vi "CO monitor TurnTable.vi"(7 "error in (no error)":errorcluster caption="에러 입력(에러 없음)", 9 "Target Offset":dbl=2.0 format="%#_13g", 10 "Instrument Manager 입력":refnum<class "Instrument Manager.lvclass">) -> (0 "error out":errorcluster caption="에러 출력", 1 "In Offset Range?":bool, 2 "Current Angle":dbl, 3 "Instrument Manager 출력":refnum<class "Instrument Manager.lvclass">)   [LabVIEW 2023, in "Instrument Manager.lvclass"]
uses:
  Instrument Manager.lvclass
  Instrument Manager.lvclass/Instrument Manager.ctl
  Module/Turn Table and Mast Control/Interface Class/Turn Table/Interface - Turn Table.lvclass
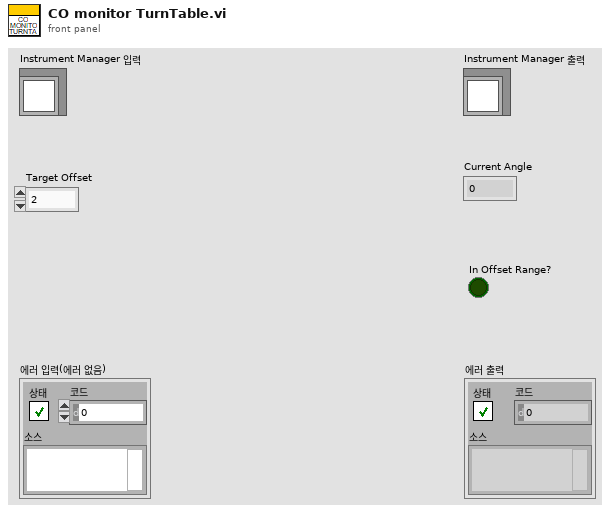
[diagram p1: front panel]
types:
  T1 = cluster{"Anritsu Call Box":refnum<class "Anritsu Call Box.lvclass">, "Spectrum Analyzer":refnum<class "Interface_Spectrum.lvclass">, "RF Switch Box":refnum<class "RF Filter Box.lvclass">, "Turn Table":refnum<class "Interface - Turn Table.lvclass">, "Mast":refnum<class "Interface - Mast.lvclass">, "3D Controller":refnum<class "Interface_3D Controller.lvclass">}
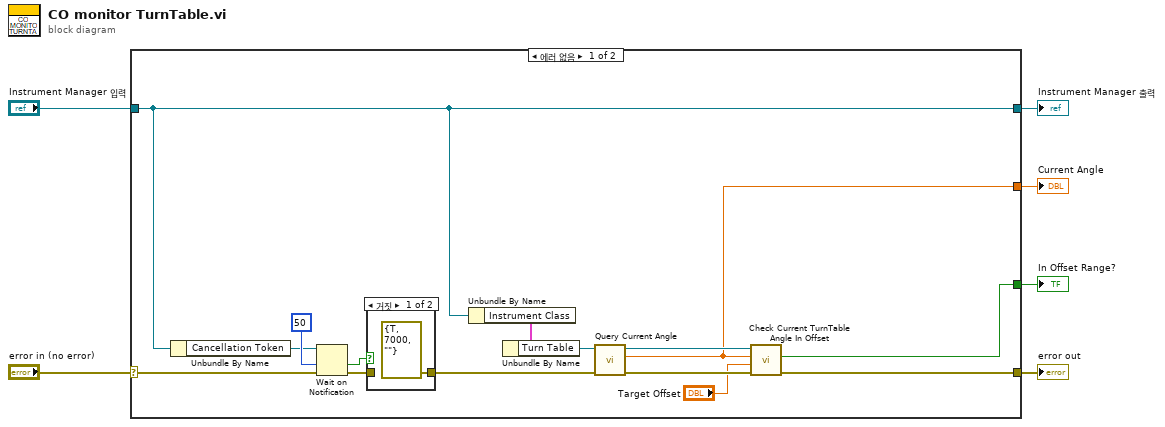
[diagram p0: block diagram]
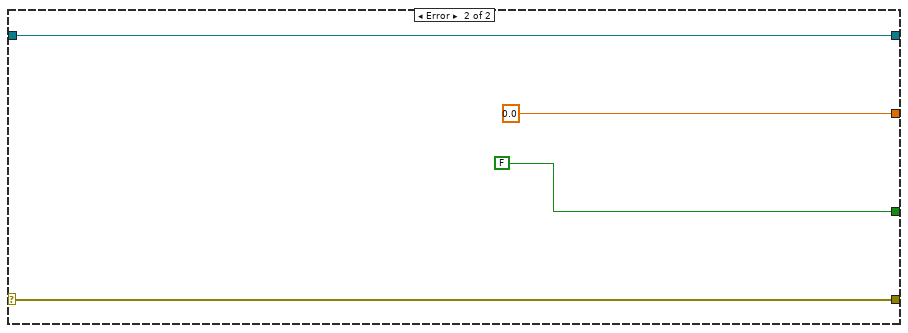
[diagram p3: hidden frame]
diagram:
  n1 = case shown="에러 없음" "error in (no error)" {
    selector: "error in (no error)" -> [w19 w27]
    tunnel: [w11 w27] -> w5
    tunnel: [w9 w26] -> w3
    tunnel: "Instrument Manager 입력" -> [w9 w26]
    tunnel: [w10 FALSE ("In Offset Range?")] -> w2
    tunnel: [w7 0.0 ("Current Angle")] -> w1
    frame No Error {
      n2 = Unbundle By Name(w9) -> ("Cancellation Token"=w8:refnum<notifier>)
      n3 = Wait on Notification(notifier=w8, timeout in ms (-1)=50 ("타임아웃(ms) (-1)"), error in (no error)=w19) -> (timed out?=w14:bool, error out=w13:errorcluster)  [unwired: 1 in, 2 out]
      n4 = case shown="거짓" w14 {
        tunnel: w13 -> [_ w23]
        tunnel: [errorcluster {"status"=TRUE, "code"=7000, "source"=""} ("error out") w23] -> w12
        frame False {
        }
        frame True {
        }
      }
      n5 = Unbundle By Name(w9) -> ("Instrument Class"=w21:T1)
      n6 = Unbundle By Name(w21) -> ("Turn Table"=w20:refnum<class "Interface - Turn Table.lvclass">)
      n7 = call-dynamic "Query Current Angle.vi"("error in (no error)"=w12, "Interface - Turn Table in"=w20) -> ("error out"=w17:errorcluster, "Current Angle"=w7:dbl, "Interface - Turn Table out"=w18:refnum<class "Interface - Turn Table.lvclass">)  [unwired: 7 in]
      n8 = call-dynamic "Check Current TurnTable Angle In Offset.vi"("error in (no error)"=w17, "Target Offset"="Target Offset", "Current Angle"=w7, "Interface - Turn Table in"=w18) -> ("error out"=w11:errorcluster, "In Offset Range?"=w10:bool)  [unwired: 5 in, 1 out]
    }
    frame Error {
    }
  }
  "error out" <- w5
  "Instrument Manager 출력" <- w3
  "In Offset Range?" <- w2
  "Current Angle" <- w1
